vi "Register Item.vi"(7 "Owner":refnum<class "UniqueName.lvclass">, 8 "error in (no error)":errorcluster, 10 "New Object Name":string, 11 "Registry in":refnum<data-value>) -> (0 "error out":errorcluster, 2 "New Node":refnum<class "UniqueName.lvclass">, 3 "Registry":refnum<data-value>)   [LabVIEW 2013, in "UniqueName.lvlib" / "NameRegistry.lvclass"]
uses:
  NameRegistry.lvclass
  UniqueNameClass/UniqueName.lvclass
  UniquenessCriteria/UniquenessCriteria.lvclass
  UniqueNameClass/Key.ctl
  StringIncrement/StringIncrement.lvclass
  RandomStringGenerator/RandomStringGenerator.lvclass
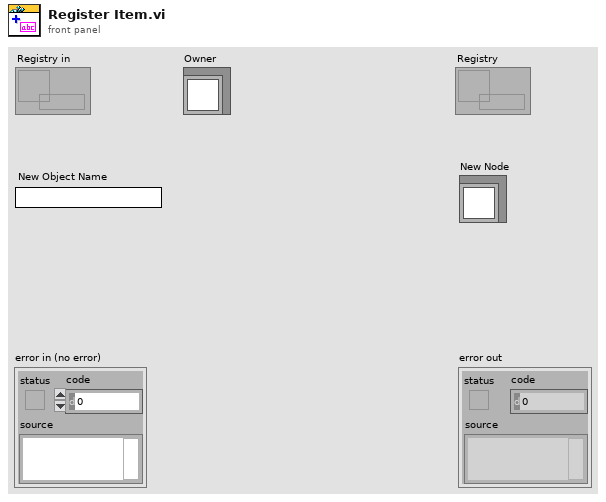
[diagram p1: front panel]
types:
  T1 = typedef "UniqueName.lvlib/UniqueName.lvclass/Key.ctl" = enum16{"Fully Qualified Name", "Unique Name", "Given Name", "Parent Fully Qualified Name", "UUID"}
  T2 = typedef "UniqueName.lvlib/UniquenessCriteria.lvclass/Criteria.ctl" = enum16{"Globally-Unique Fully Qualified Name", "Globally-Unique Name", "Universal Unique Identifier"}
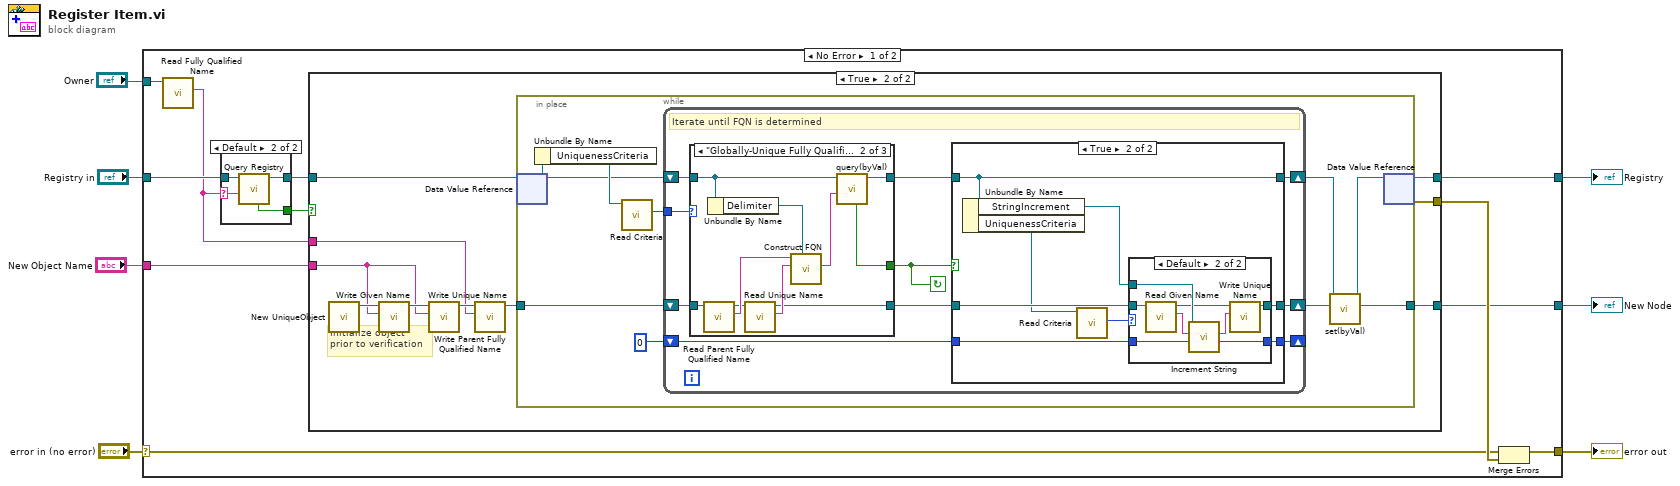
[diagram p0: block diagram]
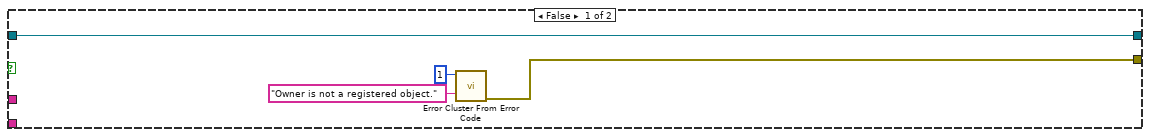
[diagram p2: hidden frame]
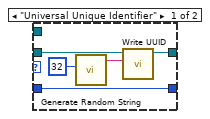
[diagram p4: hidden frame]
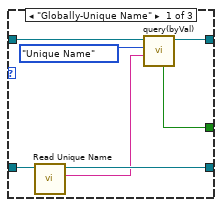
[diagram p5: hidden frame]
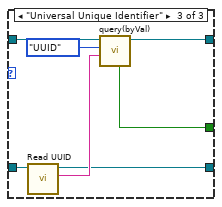
[diagram p6: hidden frame]
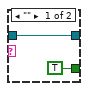
[diagram p7: hidden frame]
diagram:
  n1 = case shown="No Error" "error in (no error)" {
    selector: "error in (no error)" -> [w16 w106]
    tunnel: "Registry in" -> [w14 w107]
    tunnel: [w18 w107] -> w6
    tunnel: [w15 w106] -> w4
    tunnel: "Owner" -> [w9 _]
    tunnel: "New Object Name" -> [w11 _]
    tunnel: [w10 _] -> w2
    frame No Error {
      n2 = call "Read Fully Qualified Name.vi"("UniqueName in"=w9) -> ("Fully Qualified Name"=w8:string)  [unwired: 9 in, 1 out]
      n3 = case shown="Default" w8 {
        selector: w8 -> [_ w103]
        tunnel: w14 -> [w101 w105]
        tunnel: [w101 w104] -> w13
        tunnel: [TRUE ("found?") w102] -> w12
        frame "" {
        }
        frame Default {
          n4 = call "Query Registry.vi"("Search string"=w103, "Registry in"=w105) -> ("Registry"=w104:refnum<data-value>, "found?"=w102:bool)  [unwired: 5 in, 3 out]
        }
      }
      n5 = case shown="True" w12 {
        tunnel: [w22 w32] -> w18
        tunnel: [w20 w31] -> w17
        tunnel: w13 -> [w22 w25]
        tunnel: w11 -> [_ w27]
        tunnel: w8 -> [_ w26]
        tunnel: [_ w23] -> w10
        frame False {
          n6 = call <vilib>:"Error Cluster From Error Code.vi"("error message (\"\")"="Owner is not a registered object." ("error message (\"\")"), "error code (0)"=1) -> ("error out"=w20:errorcluster)  [unwired: 7 in]
        }
        frame True {
          # "Initialize object\nprior to verification"
          n7 = call "New UniqueObject.vi"() -> ("UniqueName out"=w30:refnum<class "UniqueName.lvclass">)  [unwired: 11 in]
          n8 = call "Write Given Name.vi"("Given Name"=w27, "UniqueName in"=w30) -> ("UniqueName out"=w28:refnum<class "UniqueName.lvclass">)  [unwired: 9 in]
          n9 = call "Write Unique Name.vi"("Unique Name"=w27, "UniqueName in"=w28) -> ("UniqueName out"=w29:refnum<class "UniqueName.lvclass">)  [unwired: 9 in]
          n10 = call "Write Parent Fully Qualified Name.vi"("Parent Fully Qualified Name"=w26, "UniqueName in"=w29) -> ("UniqueName out"=w24:refnum<class "UniqueName.lvclass">)  [unwired: 9 in]
          n11 = in-place {
            in-place-border: w24 -> [w39]
            in-place-border: [w36] -> w23
            n12 = in-place-dvr #1(w25) -> (w38:refnum<class "NameRegistry.lvclass">)  [unwired: 1 out]
            n13 = Unbundle By Name(w38) -> ("UniquenessCriteria"=w41:refnum<class "UniquenessCriteria.lvclass">)
            n14 = call "Read Criteria.vi"("UniquenessCriteria in"=w41) -> ("Criteria"=w40:T2)  [unwired: 9 in, 1 out]
            n15 = while {
              tunnel: w40 -> [w51]
              shift-right: [w49] -> w37
              shift-left: w39 -> [w48]
              shift-right: [w44] -> w34
              shift-left: w38 -> [w46]
              shift-right: [w42] -> _
              shift-left: u32 0 ("unsigned 32bit integer") -> [w43]
              stop <- w47 continue-if-true
              # "Iterate until FQN is determined"
              n16 = case shown="\"Globally-Unique Fully Qualified Name\"" w51 {
                tunnel: [w79 w86 w99] -> w47
                tunnel: w48 -> [w82 w90 w96]
                tunnel: [w81 w88 w93] -> w50
                tunnel: w46 -> [w80 w84 w97]
                tunnel: [w76 w85 w98] -> w45
                frame "Globally-Unique Name" {
                  n17 = call "Read Unique Name.vi"("UniqueName in"=w82) -> ("Unique Name"=w77:string, "UniqueName out"=w81:refnum<class "UniqueName.lvclass">)  [unwired: 9 in]
                  n18 = call "query(byVal).vi"("Search string"=w77, "Search Key (FQN)"=Key."Unique Name" ("Key (FQN)"), "Instance"=w80) -> ("Instance"=w76:refnum<class "NameRegistry.lvclass">, "found?"=w79:bool)  [unwired: 5 in, 2 out]
                }
                frame "Globally-Unique Fully Qualified Name" {
                  n19 = call "Read Parent Fully Qualified Name.vi"("UniqueName in"=w90) -> ("Parent Fully Qualified Name"=w92:string, "UniqueName out"=w89:refnum<class "UniqueName.lvclass">)  [unwired: 9 in]
                  n20 = Unbundle By Name(w84) -> ("Delimiter"=w83:refnum<class "Delimiter.lvclass">)
                  n21 = call "Read Unique Name.vi"("UniqueName in"=w89) -> ("Unique Name"=w91:string, "UniqueName out"=w88:refnum<class "UniqueName.lvclass">)  [unwired: 9 in]
                  n22 = call "Construct FQN.vi"("Delimiter"=w83, "Name"=w91, "Parent FQN"=w92) -> ("FQN"=w87:string)  [unwired: 8 in]
                  n23 = call "query(byVal).vi"("Search string"=w87, "Instance"=w84) -> ("Instance"=w85:refnum<class "NameRegistry.lvclass">, "found?"=w86:bool)  [unwired: 6 in, 2 out]
                }
                frame "Universal Unique Identifier" {
                  n24 = call "Read UUID.vi"("UniqueName in"=w96) -> ("UUID"=w94:string, "UniqueName out"=w93:refnum<class "UniqueName.lvclass">)  [unwired: 9 in]
                  n25 = call "query(byVal).vi"("Search string"=w94, "Search Key (FQN)"=Key."UUID", "Instance"=w97) -> ("Instance"=w98:refnum<class "NameRegistry.lvclass">, "found?"=w99:bool)  [unwired: 5 in, 2 out]
                }
              }
              n26 = case shown="True" w47 {
                tunnel: w50 -> [w54 w59]
                tunnel: [w54 w61] -> w49
                tunnel: w43 -> [w52 w58]
                tunnel: w45 -> [w53 w62]
                tunnel: [w53 w62] -> w44
                tunnel: [w52 w60] -> w42
                frame False {
                  # "Name already unique"
                }
                frame True {
                  n27 = Unbundle By Name(w62) -> ("StringIncrement"=w57:refnum<class "StringIncrement.lvclass">, "UniquenessCriteria"=w55:refnum<class "UniquenessCriteria.lvclass">)
                  n28 = call "Read Criteria.vi"("UniquenessCriteria in"=w55) -> ("Criteria"=w56:T2)  [unwired: 9 in, 1 out]
                  n29 = case shown="Default" w56 {
                    tunnel: [w66 w75] -> w61
                    tunnel: w57 -> [_ w73]
                    tunnel: w59 -> [w65 w72]
                    tunnel: [w67 w69] -> w60
                    tunnel: w58 -> [w67 w68]
                    frame "Universal Unique Identifier" {
                      n30 = call "Generate Random String.vi"("String Length (32)"=u32 32) -> ("Random String"=w64:string)  [unwired: 10 in]
                      n31 = call "Write UUID.vi"("UUID"=w64, "UniqueName in"=w65) -> ("UniqueName out"=w66:refnum<class "UniqueName.lvclass">)  [unwired: 9 in]
                    }
                    frame Default {
                      n32 = call "Read Given Name.vi"("UniqueName in"=w72) -> ("Given Name"=w71:string, "UniqueName out"=w70:refnum<class "UniqueName.lvclass">)  [unwired: 9 in]
                      n33 = call "Increment String.vi"("Numeric"=w68, "Input String"=w71, "StringIncrement"=w73) -> ("Incremented Numeric"=w69:u32, "Incremented String"=w74:string)  [unwired: 7 in]
                      n34 = call "Write Unique Name.vi"("Unique Name"=w74, "UniqueName in"=w70) -> ("UniqueName out"=w75:refnum<class "UniqueName.lvclass">)  [unwired: 9 in]
                    }
                  }
                }
              }
            }
            n35 = call "set(byVal).vi"("UniqueName in"=w37, "NameRegistry in"=w34) -> ("UniqueName out"=w36:refnum<class "UniqueName.lvclass">, "NameRegistry out"=w33:refnum<class "NameRegistry.lvclass">)  [unwired: 7 in, 1 out]
            n36 = in-place-dvr #1(w33) -> (w32:refnum<data-value>, w31:errorcluster)
          }
        }
      }
      n37 = Merge Errors(w16, w17) -> (w15:errorcluster)
    }
    frame Error {
    }
  }
  "error out" <- w4
  "Registry" <- w6
  "New Node" <- w2
